vi "FuncVI_Sub - File - get longest directory path.vi"(4 "path in":path) -> (1 "path out":path)   [LabVIEW 2021]
doc: "::: CalcExpress Toolkit :::\nCopyright (c) 2000-2026 Konstantin Shifershteyn. All rights reserved."
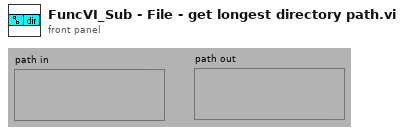
[diagram p1: front panel]
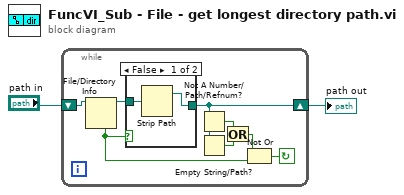
[diagram p0: block diagram]
diagram:
  n1 = while {
    shift-left: "path in" -> [w10]
    shift-right: [w7] -> w1
    stop <- w3 continue-if-true
    n2 = File/Directory Info(path=w10) -> (path out=w9:path, directory=w8:bool)  [unwired: 1 in, 5 out]
    n3 = case shown="False" w8 {
      tunnel: w9 -> [w12 w13]
      tunnel: [w11 w13] -> w7
      frame False {
        n4 = Strip Path(path=w12) -> (stripped path=w11:path)  [unwired: 1 out]
      }
      frame True {
      }
    }
    n5 = Not A Number/Path/Refnum?(number/path/refnum=w7) -> (NaN/Path/Refnum?=w5:bool)
    n6 = Empty String/Path?(string/path=w7) -> (empty?=w6:bool)
    n7 = Or(x=w5, y=w6) -> (x .or. y?=w4:bool)
    n8 = Not Or(1:w8, 2:w4) -> (0:w3:bool)
  }
  "path out" <- w1
